vi "SelectMethodsOfInterfaces.vi"(8 "error in":errorcluster, 11 "InterfacePath":T1[](array[typedef])=[{"Name(Short if no Conflicts)"="Sub_Interface1", "FullQualifierName"="Sub_Interface1.lvclass", "Description"="", "Path"=path "C:/Projects/Interface/Sub_Interface1/Sub_Interface1.lvclass", "ParentInterfaceNames(Short if no Conflitcs)"=[], "ParentInterfaceFullQualifierNames"=[], "IconPath"=path "C:/Program Files (x86)/National Instruments/LabVIEW 2020/resource/Framework/Providers/Open_GDS/icons/InterfaceBlue.png", "Methods"=[{"Name"="Add.vi", "Descriptions"="This is an Add Interface Method", "RelativePath"=path "../Add.vi", "SourceScope"=enum."public", "MustOverride"=TRUE, "VirtualFolderLocation"=["Folder"], "DynamicDispatch"=FALSE}, {"Name"="Execute.vi", "Descriptions"="", "RelativePath"=path "../Execute.vi", "SourceScope"=enum."public", "MustOverride"=TRUE, "VirtualFolderLocation"=[], "DynamicDispatch"=FALSE}], "DynamicDispatchMethod"=[]}, {"Name(Short if no Conflicts)"="Interface1", "FullQualifierName"="Interface1.lvclass", "Description"="", "Path"=path "C:/Projects/Interface/Interface1/Interface1.lvclass", "ParentInterfaceNames(Short if no Conflitcs)"=["Sub_Interface1"], "ParentInterfaceFullQualifierNames"=["Sub_Interface1.lvclass"], "IconPath"=path "C:/Program Files (x86)/National Instruments/LabVIEW 2020/resource/Framework/Providers/Open_GDS/icons/InterfaceBrown.png", "Methods"=[{"Name"="Execute2.vi", "Descriptions"="", "RelativePath"=path "../Execute2.vi", "SourceScope"=enum."public", "MustOverride"=TRUE, "VirtualFolderLocation"=[], "DynamicDispatch"=FALSE}, {"Name"="", "Descriptions"="", "RelativePath"=path "", "SourceScope"=enum."invalid scope", "MustOverride"=FALSE, "VirtualFolderLocation"=[], "DynamicDispatch"=FALSE}], "DynamicDispatchMethod"=[]}]) -> (0 "error out":errorcluster, 3 "MethodsPerInterface(Empty=>All)":cluster{"Methods":string[]}[](array[cluster]))   [LabVIEW 2020, in "InterfaceLibrary.lvlib"]
uses:
  InterfaceLibrary.lvlib
  InterfaceInfo.ctl
  LvClass_class/GDSLvClass_ClassMethodInfo.ctl
panel:
  in  "Tree":string(tree) caption="No methods selected"
  in  "Cancel":bool
  in  "Ok":bool
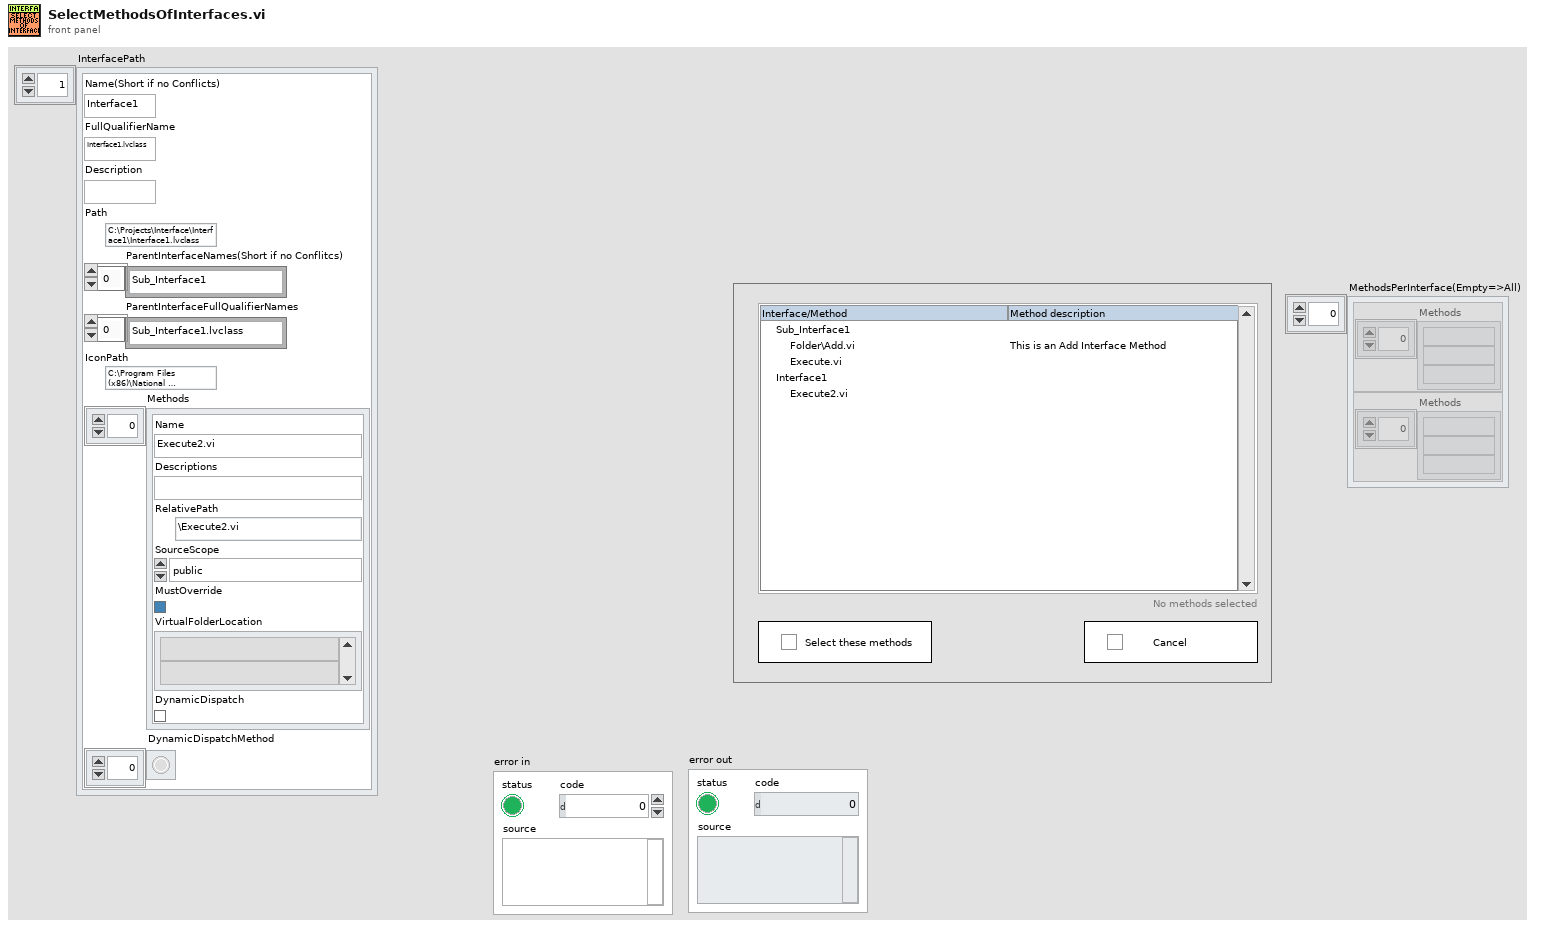
[diagram p1: front panel]
types:
  T1 = typedef "InterfaceLibrary.lvlib/InterfaceInfo.ctl" = cluster{"Name(Short if no Conflicts)":string, "FullQualifierName":string, "Description":string, "Path":path, "ParentInterfaceNames(Short if no Conflitcs)":string[], "ParentInterfaceFullQualifierNames":string[], "IconPath":path, "Methods":T2[], "DynamicDispatchMethod":bool[]}
  T2 = typedef "GDSLvClass_ClassMethodInfo.ctl" = cluster{"Name":string, "Descriptions":string, "RelativePath":path, "SourceScope":enum32{"invalid scope", "public", "private", "protected", "community"}, "MustOverride":bool, "VirtualFolderLocation":string[], "DynamicDispatch":bool}
  T3 = typedef "LVPoint32TypeDef.ctl" = cluster{"Horizontal":i32, "Vertical":i32}
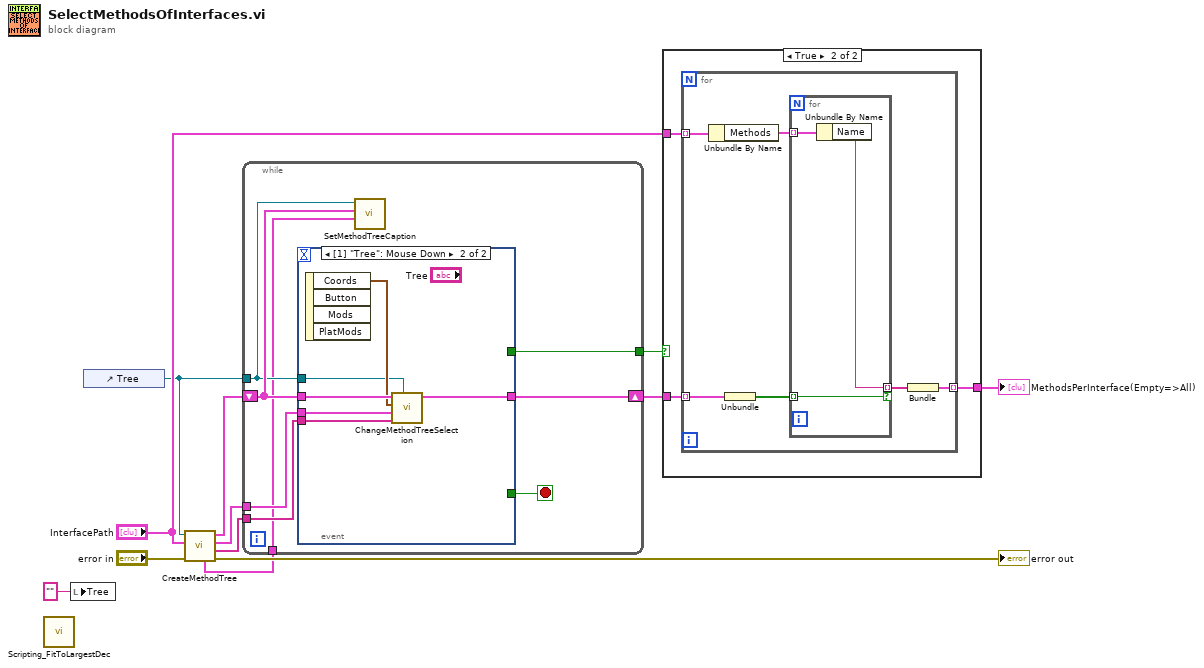
[diagram p0: block diagram]
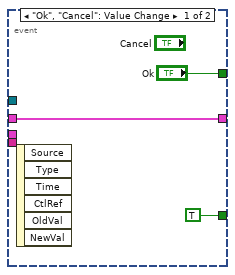
[diagram p2: hidden frame]
diagram:
  n1 = call "Scripting_FitToLargestDec.vi"() -> ()  [unwired: 6 in, 2 out]
  n2 = local write "Tree"("" ("Tree")) -> ()
  n3 = control-ref of="Tree"() -> (w2:refnum<vi>)
  n4 = call "CreateMethodTree.vi"("error in (no error)"="error in", "InterfacePath"="InterfacePath", "TreeControlRef"=w2) -> ("error out"=→"error out":errorcluster, "InterfacesTag"=w10:string[], "MethodsTagPerInterfaces"=w9:cluster{"Array":string[]}[], "MethodsSelectedPerInterface"=w8:cluster{"Array":bool[]}[], "MethodsDisabledPerInterface"=w1:cluster{"Array":bool[]}[])  [unwired: 4 in]
  n5 = while {
    tunnel: w10 -> [w19]
    tunnel: w9 -> [w18]
    shift-right: [w16] -> w6
    shift-left: w8 -> [w17]
    tunnel: [w15] -> w7
    tunnel: w2 -> [w14]
    tunnel: w1 -> [w13]
    stop <- w20 stop-if-true
    n6 = event shown="[1] \"Tree\": Mouse Down" {
      selector: _ -> [_ _]
      dyn-events: _ -> [_ _]
      timeout: _ -> [_ _]
      tunnel: [TRUE _] -> w20
      tunnel: w19 -> [_ w25]
      tunnel: w18 -> [_ w29]
      tunnel: w17 -> [w22 w27]
      tunnel: [w22 w28] -> w16
      tunnel: ["Ok" _] -> w15
      tunnel: w14 -> [_ w24]
      event "Ok", "Cancel": Value Change {
        n7 = event-data() -> ()  [unwired: 1 in, 6 out]
      }
      event "Tree": Mouse Down {
        n8 = event-data() -> ("Coords"=w26:T3)  [unwired: 1 in, 3 out]
        n9 = call "ChangeMethodTreeSelection.vi"("TreeControl in"=w24, "Interfaces"=w25, "MethodsPerInterfaces"=w29, "MouseClickCoordinates"=w26, "SelectedMethodsIn"=w27) -> ("SelectedMethodsOut"=w28:cluster{"Array":bool[]}[])  [unwired: 6 in]
      }
    }
    n10 = call "SetMethodTreeCaption.vi"("MethodsDisabledPerInt"=w13, "MethodsSelectedPerInt"=w17, "TreeControl in"=w14) -> ()  [unwired: 8 in, 1 out]
  }
  n11 = case shown="True" w7 {
    tunnel: w6 -> [_ w32]
    tunnel: "InterfacePath" -> [_ w31]
    tunnel: [_ w30] -> w4
    frame False {
    }
    frame True {
      n12 = for {
        tunnel: w32 -> [w38] mode=indexing
        tunnel: w31 -> [w37] mode=indexing
        tunnel: [w33] -> w30 mode=indexing
        n13 = Unbundle By Name(w37) -> ("Methods"=w36:T2[])
        n14 = Unbundle(w38) -> ("Array"=w35:bool[])
        n15 = for {
          tunnel: w36 -> [w41] mode=indexing
          tunnel: w35 -> [w39] mode=indexing
          tunnel: [w40] -> w34 mode=indexing if=w39
          n16 = Unbundle By Name(w41) -> ("Name"=w40:string)
        }
        n17 = Bundle(w34) -> (w33:cluster{string[]})  [unwired: 1 in]
      }
    }
  }
  "MethodsPerInterface(Empty=>All)" <- w4
